vi "VIH - CHM Project - Write TOC File - Add HTML Files.vi"(7 "Base Dir Path":path, 8 "error in":errorcluster, 9 "Project Files":T2, 11 "HTML in":string) -> (0 "error out":errorcluster, 3 "HTML out":string)   [LabVIEW 2014]
doc: "::: VI Helpeks :::\nCopyright (c) 2000-2026 Konstantin Shifershteyn. All rights reserved."
uses:
  _VIH HelpGen - Palette.llb/VIH HelpGen Typedef - Palette - Item Type Enum.ctl
panel:
  # "VI Helpeks\nCopyright (c) 2012-2026 Konstantin Shifershteyn"
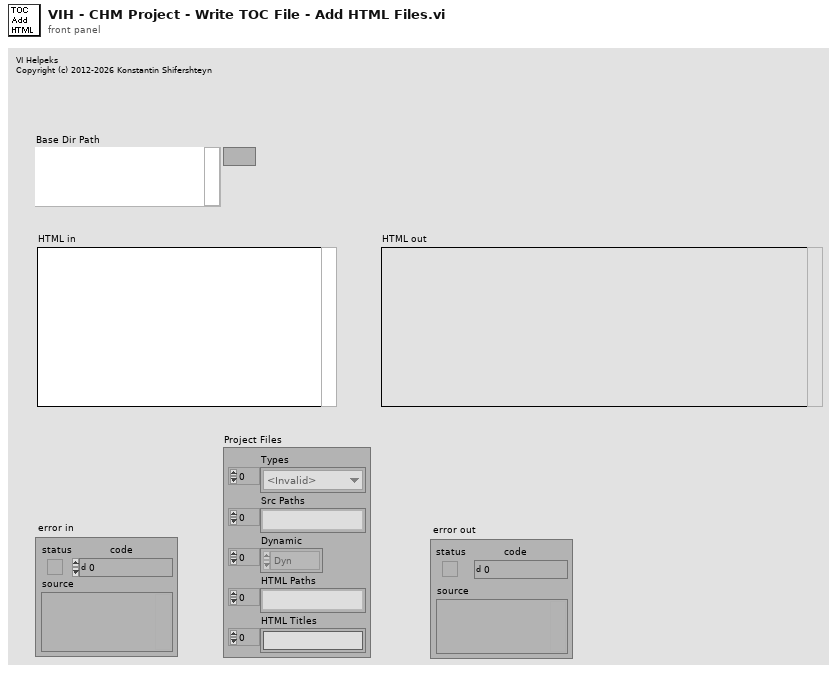
[diagram p1: front panel]
types:
  T1 = typedef "VIH HelpGen Typedef - Palette - Item Type Enum.ctl" = enum32{"<Invalid>", "<unknown>", "VI", "Menu", "LV Func", "Express VI", "Poly VI", "CTL", "HTML"}
  T2 = cluster{"Types":T1[], "Src Paths":path[], "Dynamic":enum16{"Dyn", "Stat", "Both"}[], "HTML Paths":path[], "HTML Titles":string[]}
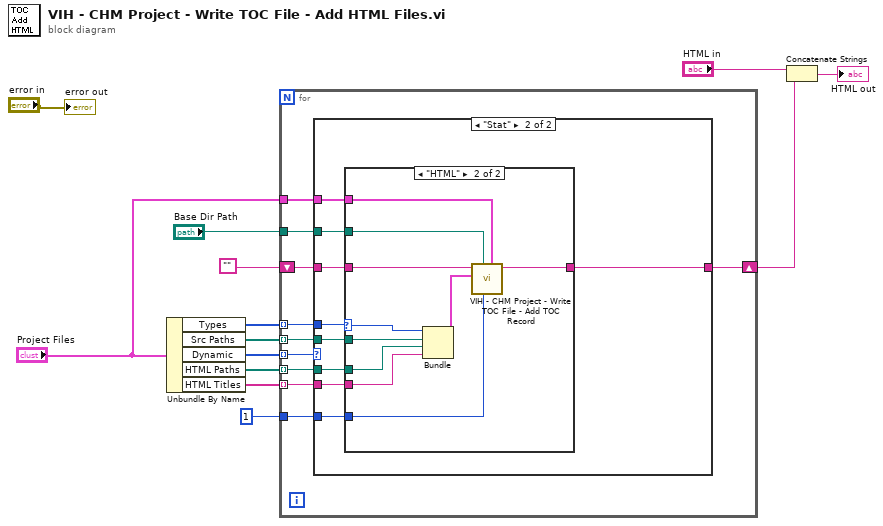
[diagram p0: block diagram]
diagram:
  n1 = Unbundle By Name("Project Files") -> ("Types"=w10:T1[], "Src Paths"=w11:path[], "Dynamic"=w13:enum16{"Dyn", "Stat", "Both"}[], "HTML Paths"=w9:path[], "HTML Titles"=w7:string[])
  n2 = for {
    tunnel: w13 -> [w23] mode=indexing
    shift-right: [w20] -> w2
    shift-left: "" -> [w22]
    tunnel: "Project Files" -> [w21]
    tunnel: w11 -> [w19] mode=indexing
    tunnel: w10 -> [w18] mode=indexing
    tunnel: w9 -> [w17] mode=indexing
    tunnel: "Base Dir Path" -> [w16]
    tunnel: w7 -> [w15] mode=indexing
    tunnel: 1 ("Level") -> [w14]
    n3 = case shown="\"Stat\"" w23 {
      tunnel: w22 -> [w24 w33]
      tunnel: w21 -> [_ w32]
      tunnel: [w24 w31] -> w20
      tunnel: w19 -> [_ w29]
      tunnel: w18 -> [_ w26]
      tunnel: w17 -> [_ w28]
      tunnel: w16 -> [_ w30]
      tunnel: w15 -> [_ w27]
      tunnel: w14 -> [_ w25]
      frame Default {
      }
      frame "Stat" {
        n4 = case shown="\"HTML\"" w26 {
          selector: w26 -> [_ w35]
          tunnel: w33 -> [w34 w44]
          tunnel: w32 -> [_ w43]
          tunnel: [w34 w42] -> w31
          tunnel: w30 -> [_ w41]
          tunnel: w29 -> [_ w40]
          tunnel: w28 -> [_ w39]
          tunnel: w27 -> [_ w38]
          tunnel: w25 -> [_ w36]
          frame Default {
          }
          frame "HTML" {
            n5 = Bundle("Item/File Type"=w35, w40, w39, w38) -> (w37:cluster{"Item/File Type":T1, path, path, string})  [unwired: 1 in]
            n6 = call "VIH - CHM Project - Write TOC File - Add TOC Record.vi"("Project Files"=w43, "Level"=w36, "Base Dir Path"=w41, "File Params"=w37, "HTML in"=w44) -> ("HTML out"=w42:string)  [unwired: 6 in]
          }
        }
      }
    }
  }
  n7 = Concatenate Strings("HTML in", w2) -> (→"HTML out":string)
  "error out" <- "error in"
